vi "Duplicate Case Structure Frames.vi"(8 "error in (no error)":errorcluster, 10 "Frame Names":string[](array[string]), 11 "CaseStructure in":refnum<vi>) -> (0 "error out":errorcluster, 2 "Case Frames[]":refnum<vi>[](array[refnum]), 3 "CaseStructure out":refnum<vi>)   [LabVIEW 2019, in "gRPC Template Creation Utility.lvlib"]
uses:
  gRPC Template Creation Utility.lvlib
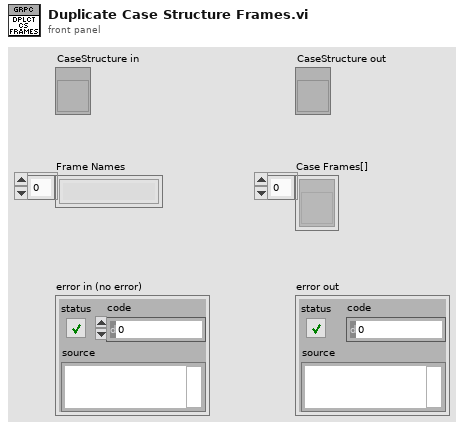
[diagram p1: front panel]
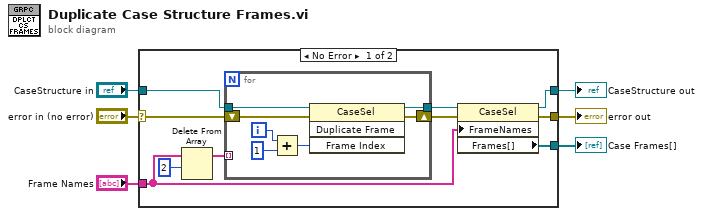
[diagram p0: block diagram]
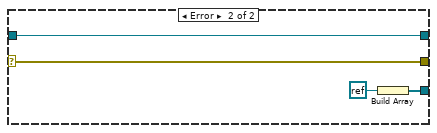
[diagram p2: hidden frame]
diagram:
  n1 = case shown="No Error" "error in (no error)" {
    selector: "error in (no error)" -> [w8 w27]
    tunnel: [w15 w24] -> w6
    tunnel: [w14 w27] -> w5
    tunnel: "Frame Names" -> [w13 _]
    tunnel: [w11 w25] -> w3
    tunnel: "CaseStructure in" -> [w7 w24]
    frame No Error {
      n2 = Delete From Array(array=w13, length=2) -> (array with subset deleted=w12:string[])  [unwired: 1 in, 1 out]
      n3 = for {
        tunnel: w7 -> [w23]
        tunnel: [w21] -> w16
        shift-right: [w20] -> w10
        shift-left: w8 -> [w22]
        tunnel: w12 -> [_] mode=indexing
        i -> [w19]
        n4 = Add(x=w19, y=1) -> (x+y=w18:i32)
        n5 = invoke class="CaseSel" method="Duplicate Frame"(reference=w23, error in=w22, "Frame Index"=w18) -> (reference out=w21:refnum<vi>, error out=w20:errorcluster)  [unwired: 1 in, 2 out]
      }
      n6 = property class="CaseSel"(reference=w16, error in=w10, "FrameNames"=w13) -> (reference out=w15:refnum<vi>, error out=w14:errorcluster, "Frames[]"=w11:refnum<vi>[])
    }
    frame Error {
      n7 = Build Array(refnum<k0> refnum) -> (w25:refnum<k0>[])
    }
  }
  "error out" <- w5
  "CaseStructure out" <- w6
  "Case Frames[]" <- w3
